vi "lvgit status.vi"(8 "error in":errorcluster, 11 "path":path) -> (0 "error out":errorcluster)   [LabVIEW 2017]
panel:
  out "Staged Files":string[](array[string])
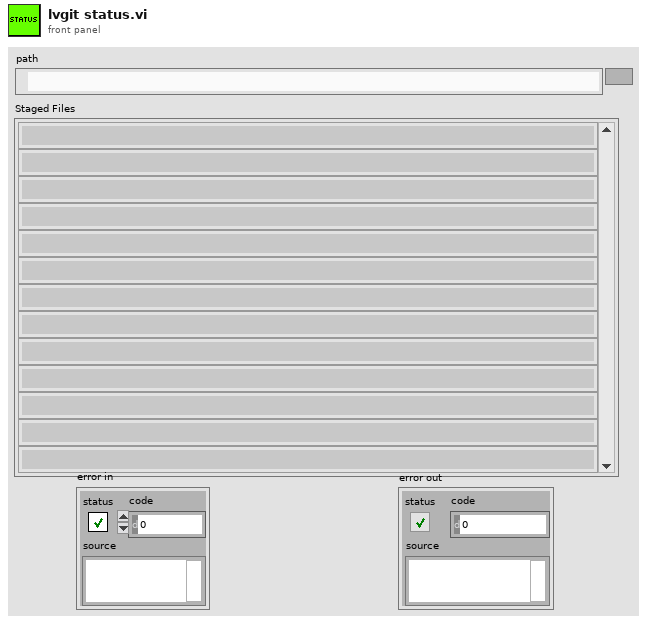
[diagram p1: front panel]
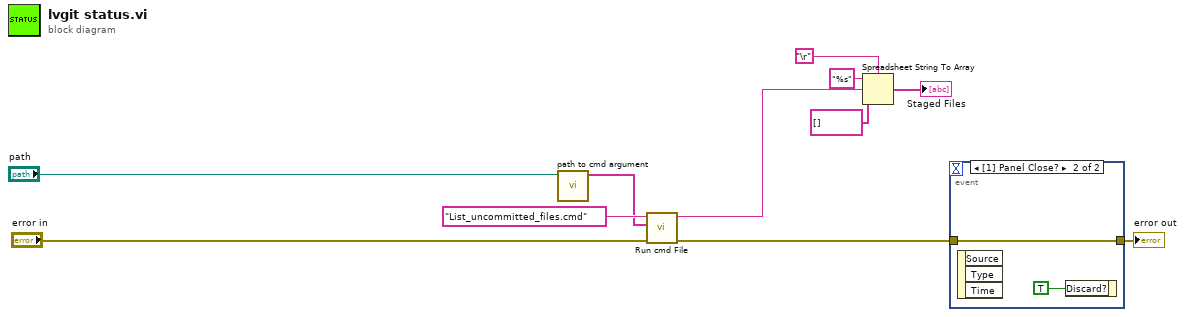
[diagram p0: block diagram]
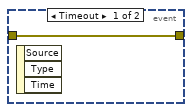
[diagram p2: hidden frame]
diagram:
  n1 = call "path to cmd argument.vi"("path"="path") -> ("Array"=w9:string[])  [unwired: 10 in]
  n2 = call "Run cmd File.vi"("Error in"="error in", "args"=w9, "name or relative path"="List_uncommitted_files.cmd") -> ("Error out"=w6:errorcluster, "standard output"=w5:string)  [unwired: 6 in, 1 out]
  n3 = Spreadsheet String To Array(delimiter (Tab)="\r", format string="%s", spreadsheet string=w5, array type (2D Dbl)=string[] [] ("Array of Strings")) -> (array=→"Staged Files":string[])
  n4 = event shown="[1] Panel Close?" {
    selector: _ -> [_ _]
    dyn-events: _ -> [_ _]
    timeout: _ -> [_ _]
    tunnel: w6 -> [w12 w14]
    tunnel: [w12 w14] -> w11
    event Timeout {
      n5 = event-data() -> ()  [unwired: 1 in, 3 out]
    }
    event Panel Close? {
      n6 = event-data() -> ()  [unwired: 1 in, 3 out]
      n7 = event-data("Discard?"=TRUE) -> ()  [unwired: 1 in, 1 out]
    }
  }
  "error out" <- w11
